vi "Read E-Series File Names.vi"(8 "error in (no error)":errorcluster, 11 "E-Series File":path) -> (0 "error out":errorcluster, 3 "E-Series File Names":T1)   [LabVIEW 2018, in "E-Series Reader.lvlib"]
doc: "Reads the file names of the E-Series from the INI configuration file.\n\nThe VI receives the <b>INI File</b> name and reads the configuration sections and their associated keys. It retrieves the value of the <b>Filename</b> key from each section and builds an array containing the E-Series file names.\n\nThe VI returns the resulting array through <b>E-Series File Names</b>. This array is intended to be used by <b>Read E-Series.vi</b> to load the E-Series data.\n\nThe VI propagates errors through its <b>error in</b> and <b>error out</b> terminals."
uses:
  E-Series Reader.lvlib
  E-Series File Names--array.ctl
  <vilib>/Utility/config.llb/Read Key (String).vi
  <vilib>/Utility/config.llb/NI_LVConfig.lvlib
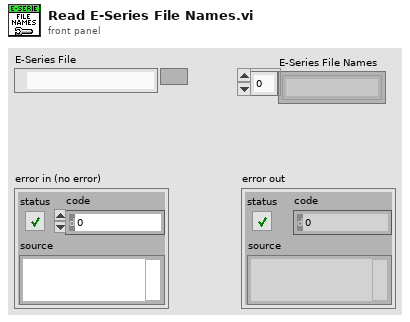
[diagram p1: front panel]
types:
  T1 = typedef "E-Series Reader.lvlib/E-Series File Names--array.ctl" = string[]
  T2 = typedef "NI_LVConfig.lvlib/Config Data RefNum.ctl" = refnum<k1>
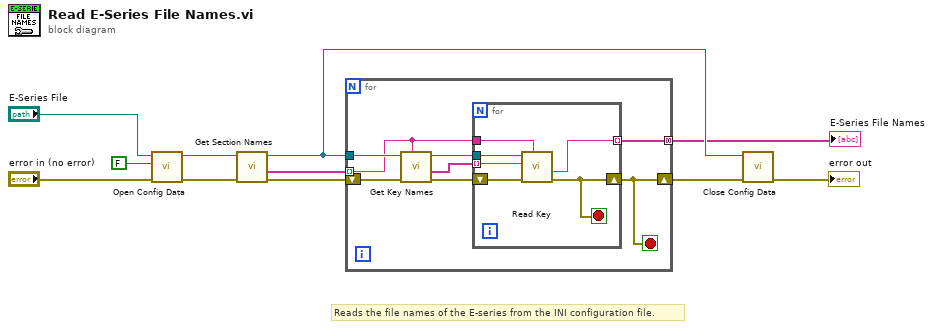
[diagram p0: block diagram]
diagram:
  # "Reads the file names of the E-series from the INI configuration file."
  n1 = call <vilib>:"Open Config Data.vi"("error in (no error)"="error in (no error)", "create file if necessary (T)"=FALSE, "configuration file path"="E-Series File") -> ("error out"=w10:errorcluster, "refnum"=w8:T2)  [unwired: 6 in, 1 out]
  n2 = call <vilib>:"Get Section Names.vi"("error in (no error)"=w10, "refnum"=w8) -> ("error out"=w9:errorcluster, "section names"=w2:string[], "refnum out"=w5:T2)  [unwired: 7 in]
  n3 = for {
    shift-right: [w12] -> w4
    shift-left: w9 -> [w19]
    tunnel: w2 -> [w16] mode=indexing
    tunnel: w5 -> [w18]
    tunnel: [w14] -> w3 mode=concatenating
    stop <- w12 stop-if-true
    n4 = call <vilib>:"Get Key Names.vi"("section"=w16, "error in (no error)"=w19, "refnum"=w18) -> ("error out"=w17:errorcluster, "key names"=w15:string[], "refnum out"=w13:T2)  [unwired: 5 in, 1 out]
    n5 = for {
      shift-right: [w20] -> w12
      shift-left: w17 -> [w25]
      tunnel: w16 -> [w24]
      tunnel: w15 -> [w23] mode=indexing
      tunnel: [w22] -> w14 mode=indexing
      tunnel: w13 -> [w21]
      stop <- w20 stop-if-true
      n6 = call-poly <vilib>:"Read Key.vi"("section"=w24, "error in (no error)"=w25, "key"=w23, "refnum"=w21) -> ("error out"=w20:errorcluster, "value"=w22:string)  [unwired: 4 in, 2 out]
    }
  }
  "E-Series File Names" <- w3
  n7 = call <vilib>:"Close Config Data.vi"("error in (no error)"=w4, "refnum"=w5) -> ("error out"=→"error out":errorcluster)  [unwired: 8 in, 1 out]
